vi "FuncVI-vhConfCx.vi"(5 "InstanceRef":T2, 9 "arg list":T1[](array[typedef]) {"num" format="%.2f"}) -> (0 "error out":bool, 3 "result":T1 {"num" format="%.2f"})   [LabVIEW 2021]
doc: "::: CalcExpress Toolkit :::\nCopyright (c) 2000-2026 Konstantin Shifershteyn. All rights reserved."
uses:
  cetypes.llb/CalcExpress Function Argument Info.ctl
  cetypes.llb/CalcExpress Instance RefNum.ctl
panel:
  in  "max arg num":i32=8
  in  "min arg num":i32=1
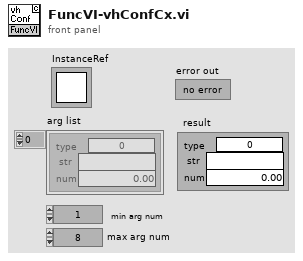
[diagram p1: front panel]
types:
  T1 = typedef "CalcExpress Function Argument Info.ctl" = cluster{"type":u32, "str":string, "num":dbl}
  T2 = typedef "CalcExpress Instance RefNum.ctl" = refnum<k1>
  T3 = enum32{"String", "DBL Number", "identifier", "1D Array of DBL", "2D Array of DBL", "CDB Number", "1D Array of CDB", "2D Array of CDB", "1D Array of String", "2D Array of String", "Unknown data type"}
  T4 = cluster{"index":i32, "data type":enum32{"String", "DBL Number", "identifier", "1D Array of DBL", "2D Array of DBL", "CDB Number", "1D Array of CDB", "2D Array of CDB", "1D Array of String", "2D Array of String", "Unknown data type"}, "default num":dbl, "default str":string}[]
  T5 = enum32{"nop", "create", "destroy", "reset", "get info", "config", "create_wrid"}
  T6 = cluster{"num list[0]":dbl, "num list[1]":dbl, "num list[2]":dbl, "num list[3]":dbl, "num list[4]":dbl, "num list[5]":dbl, "num list[6]":dbl, "num list[7]":dbl}
  T7 = typedef "VarMan Variable Context Handle.ctl" = i32
  T8 = cluster{u32, "num list[5]":dbl, "num list[6]":dbl, "num list[7]":dbl}
  T9 = cluster{"data type":enum32{"String", "DBL Number", "identifier", "1D Array of DBL", "2D Array of DBL", "CDB Number", "1D Array of CDB", "2D Array of CDB", "1D Array of String", "2D Array of String", "Unknown data type"}, string, dbl}
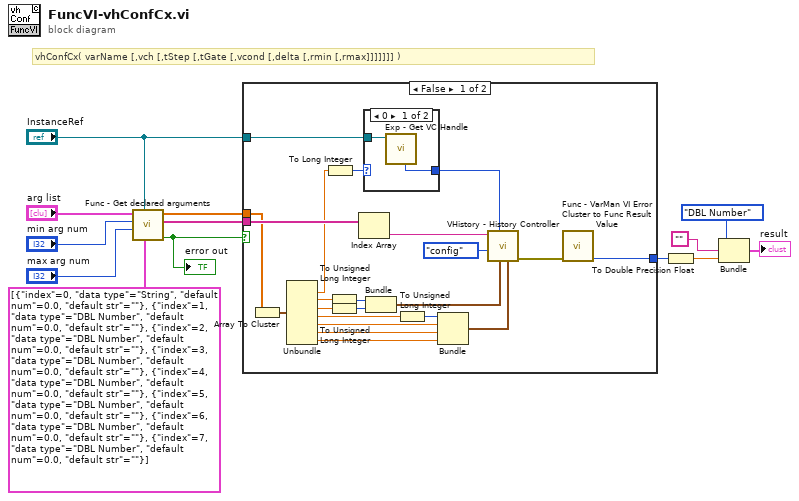
[diagram p0: block diagram]
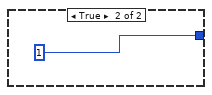
[diagram p3: hidden frame]
diagram:
  # "vhConfCx( varName [,vch [,tStep [,tGate [,vcond [,delta [,rmin [,rmax]]]]]]] )"
  n1 = call "Func - Get declared arguments.vi"("arg descriptors"=T4 [{"index"=0, "data type"=enum."String", "default num"=0.0, "default str"=""}, {"index"=1, "data type"=enum."DBL Number", "default num"=0.0, "default str"=""}, {"index"=2, "data type"=enum."DBL Number", "default num"=0.0, "default str"=""}, {"index"=3, "data type"=enum."DBL Number", "default num"=0.0, "default str"=""}, {"index"=4, "data type"=enum."DBL Number", "default num"=0.0, "default str"=""}, {"index"=5, "data type"=enum."DBL Number", "default num"=0.0, "default str"=""}, {"index"=6, "data type"=enum."DBL Number", "default num"=0.0, "default str"=""}, {"index"=7, "data type"=enum."DBL Number", "default num"=0.0, "default str"=""}], "InstanceRef"="InstanceRef", "max arg num"="max arg num", "min arg num"="min arg num", "arg list"="arg list") -> ("error out"=w12:bool, "str list"=w8:string[], "num list"=w1:dbl[])  [unwired: 3 in, 1 out]
  "error out" <- w12
  n2 = case shown="False" w12 {
    tunnel: w1 -> [w29 _]
    tunnel: w8 -> [w35 _]
    tunnel: [w14 1 ("code")] -> w7
    tunnel: "InstanceRef" -> [w33 _]
    frame False {
      n3 = Array To Cluster(array=w29) -> (cluster=w30:T6)
      n4 = Unbundle(w30) -> ("num list[1]"=w17:dbl, "num list[2]"=w18:dbl, "num list[3]"=w19:dbl, "num list[4]"=w20:dbl, "num list[5]"=w23:dbl, "num list[6]"=w24:dbl, "num list[7]"=w25:dbl)  [unwired: 1 out]
      n5 = To Long Integer(number=w17) -> (32bit integer=w31:i32)
      n6 = To Unsigned Long Integer(number=w18) -> (unsigned 32bit integer=w28:u32)
      n7 = To Unsigned Long Integer(number=w19) -> (unsigned 32bit integer=w27:u32)
      n8 = Index Array(array=w35) -> (element=w34:string)  [unwired: 1 in]
      n9 = case shown="0" w31 {
        selector: w31 -> [_ w38]
        tunnel: w33 -> [w37 _]
        tunnel: [w36 w38] -> w32
        frame 0 {
          n10 = call "Exp - Get VC Handle.vi"("InstanceRef"=w37) -> ("VC Handle"=w36:T7)  [unwired: 5 in, 3 out]
        }
        frame Default {
        }
      }
      n11 = Bundle(w28, w27) -> (w26:cluster{u32, u32})  [unwired: 1 in]
      n12 = To Unsigned Long Integer(number=w20) -> (unsigned 32bit integer=w21:u32)
      n13 = Bundle(w21, "num list[5]"=w23, "num list[6]"=w24, "num list[7]"=w25) -> (w22:T8)  [unwired: 1 in]
      n14 = call "VHistory - History Controller.vi"("value condition"=w22, "time conditions"=w26, "VC Handle"=w32, "cmd (nop:default)"=T5."config", "name_spec"=w34) -> ("error out"=w15:errorcluster)  [unwired: 3 in, 3 out]
      n15 = call "Func - VarMan VI Error Cluster to Func Result Value.vi"("VarMan VI error in"=w15) -> ("CE Function Result Value"=w14:i32)  [unwired: 10 in]
    }
    frame True {
    }
  }
  n16 = To Double Precision Float(number=w7) -> (double precision float=w6:dbl)
  n17 = Bundle("data type"=T3."DBL Number", "", w6) -> (→"result":T9)  [unwired: 1 in]
